vi "Test MQTT-3.1.0-2.vi"(8 "error in (no error)":errorcluster, 11 "Connection Config":refnum<class "Connection.lvclass">) -> (0 "error out":errorcluster, 3 "Connection Config dup":refnum<class "Connection.lvclass">)   [LabVIEW 2013]
uses:
  <vilib>/LabVIEW Open Source Project/MQTT Control Packets/Control Packets/ControlPacket/ControlPacket.lvclass
  <vilib>/addons/_JKI Toolkits/Caraya/classes/Test/Test.lvclass
  <vilib>/addons/_JKI Toolkits/Caraya/classes/Assert/Assert.lvclass
  <vilib>/LabVIEW Open Source Project/MQTT Control Packets/Control Packets/CONNECT/CONNECT.lvclass
  <vilib>/LabVIEW Open Source Project/Connection/Connection/Connection.lvclass
  <vilib>/LabVIEW Open Source Project/MQTT Connection/MQTT_Connection/Connection/Connection.lvclass
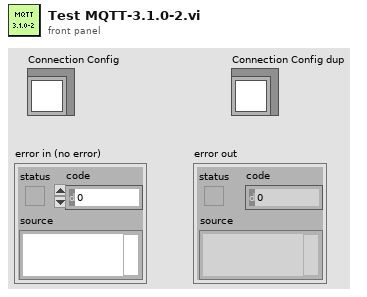
[diagram p1: front panel]
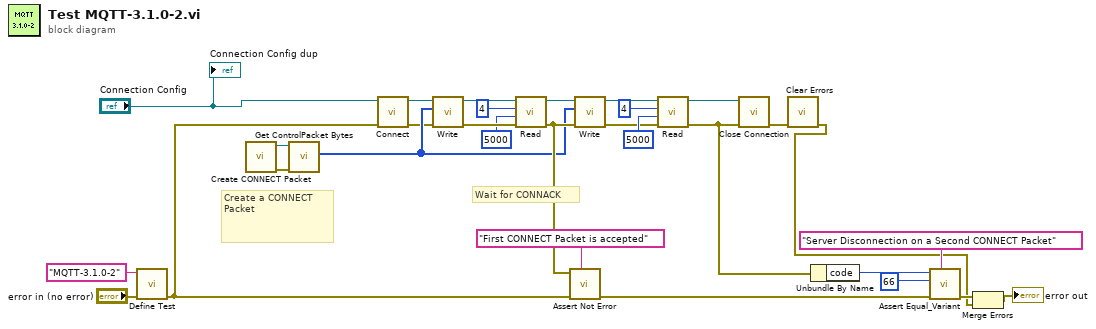
[diagram p0: block diagram]
diagram:
  # "Wait for CONNACK"
  # "Create a CONNECT Packet"
  n1 = call <vilib>:"Define Test.vi"("error in (no error)"="error in (no error)", "Label (VI Title)"="MQTT-3.1.0-2") -> ("error out"=w2:errorcluster)  [unwired: 9 in]
  n2 = call <vilib>:"Create CONNECT Packet.vi"() -> ("error out"=w16:errorcluster, "CONNECT"=w17:refnum<class "CONNECT.lvclass">)  [unwired: 9 in, 1 out]
  n3 = call <vilib>:"Get ControlPacket Bytes.vi"("error in (no error)"=w16, "ControlPacket"=w17) -> ("Bytes Stream"=w5:u8[])  [unwired: 6 in, 3 out]
  n4 = call <vilib>:"Connect.vi"("error in (no error)"=w2, "Connection in"="Connection Config") -> ("error out"=w3:errorcluster, "Connection out"=w4:refnum<class "Connection.lvclass">)  [unwired: 8 in]
  n5 = call <vilib>:"Write.vi"("error in (no error)"=w3, "Bytes"=w5, "Connection in"=w4) -> ("error out"=w29:errorcluster, "Connection"=w30:refnum<class "Connection.lvclass">)  [unwired: 7 in]
  n6 = call <vilib>:"Read.vi"("error in (no error)"=w29, "timeout (2000 ms)"=5000 ("timeout ms (25000)"), "bytes to read (100)"=4 ("bytes to read"), "TCPConnection in"=w30) -> ("error out"=w8:errorcluster, "TCPConnection out"=w9:refnum<class "Connection.lvclass">)  [unwired: 3 in, 3 out]
  n7 = call <vilib>:"Assert Not Error.vi"("Label"="First CONNECT Packet is accepted", "error in (no error)"=w2, "Not Error?"=w8) -> ("error out"=w15:errorcluster)  [unwired: 8 in]
  n8 = call <vilib>:"Write.vi"("error in (no error)"=w8, "Bytes"=w5, "Connection in"=w9) -> ("error out"=w11:errorcluster, "Connection"=w10:refnum<class "Connection.lvclass">)  [unwired: 7 in]
  n9 = call <vilib>:"Read.vi"("error in (no error)"=w11, "timeout (2000 ms)"=5000 ("timeout ms (25000)"), "bytes to read (100)"=4 ("bytes to read"), "TCPConnection in"=w10) -> ("error out"=w7:errorcluster, "TCPConnection out"=w6:refnum<class "Connection.lvclass">)  [unwired: 3 in, 3 out]
  n10 = call <vilib>:"Close Connection.vi"("error in (no error)"=w7, "Connection in"=w6) -> ("error out"=w22:errorcluster)  [unwired: 8 in, 1 out]
  n11 = call <vilib>:"Clear Errors.vi"("error in (no error)"=w22) -> ("error out"=w18:errorcluster)  [unwired: 6 in]
  n12 = Unbundle By Name(w7) -> ("code"=w24:i32)
  n13 = call <vilib>:"Assert Equal_Variant.vi"("Label"="Server Disconnection on a Second CONNECT Packet", "error in (no error)"=w15, "Y"=66 ("code"), "X"=w24) -> ("error out"=w27:errorcluster)  [unwired: 7 in]
  n14 = Merge Errors(w27, w18) -> (→"error out":errorcluster)
  "Connection Config dup" <- "Connection Config"
